vi "TimeSyncServ_GetAll.vi"() -> (0 "PV_TimeSyncStopServ":bool, 1 "PV_TimeSyncLastSentTime":i64, 2 "PV_TimeSyncLastRcvTim":i64, 3 "PV_TimeSyncLastRcvId":i8, 4 "PV_TimeSyncLoopCount":i32, 5 "PV_TimeSyncLastRcvVer":i8, 6 "PV_TimeSyncServWriteErr":bool, 7 "PV_TimeSyncServRcvIP":u32, 8 "PV_TimeSyncServReadErr":bool, 11 "PV_TimeSyncServLastSrcPort":u32)   [LabVIEW 2019, in "PhotonVisionLib.lvlib"]
doc: "Get information on photonvision time sync server.\n\nInputs:\n - <None>\n\nOutputs:\n - <Various>"
uses:
  PhotonVisionLib.lvlib
  PhotonVision_Globals.vi
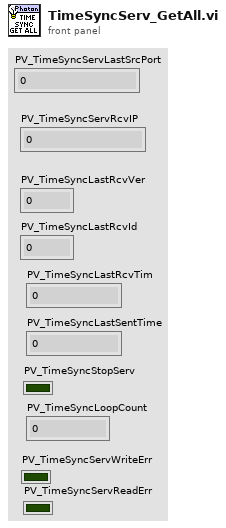
[diagram p1: front panel]
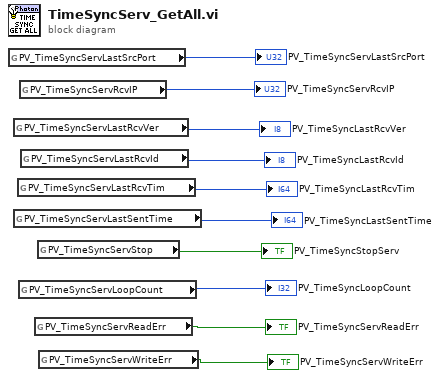
[diagram p0: block diagram]
diagram:
  n1 = global read "PhotonVision_Globals.vi" "PV_TimeSyncServLastSrcPort"() -> (→"PV_TimeSyncServLastSrcPort":u32)
  n2 = global read "PhotonVision_Globals.vi" "PV_TimeSyncServLastRcvVer"() -> (→"PV_TimeSyncLastRcvVer":i8)
  n3 = global read "PhotonVision_Globals.vi" "PV_TimeSyncServLastSentTime"() -> (→"PV_TimeSyncLastSentTime":i64)
  n4 = global read "PhotonVision_Globals.vi" "PV_TimeSyncServLastRcvTim"() -> (→"PV_TimeSyncLastRcvTim":i64)
  n5 = global read "PhotonVision_Globals.vi" "PV_TimeSyncServLoopCount"() -> (→"PV_TimeSyncLoopCount":i32)
  n6 = global read "PhotonVision_Globals.vi" "PV_TimeSyncServRcvIP"() -> (→"PV_TimeSyncServRcvIP":u32)
  n7 = global read "PhotonVision_Globals.vi" "PV_TimeSyncServLastRcvId"() -> (→"PV_TimeSyncLastRcvId":i8)
  n8 = global read "PhotonVision_Globals.vi" "PV_TimeSyncServReadErr"() -> (→"PV_TimeSyncServReadErr":bool)
  n9 = global read "PhotonVision_Globals.vi" "PV_TimeSyncServStop"() -> (→"PV_TimeSyncStopServ":bool)
  n10 = global read "PhotonVision_Globals.vi" "PV_TimeSyncServWriteErr"() -> (→"PV_TimeSyncServWriteErr":bool)
